vi "GV-GetLegendRange.vi"(8 "error in (no error)":errorcluster, 9 "Coords":T1, 11 "Gviewer in":refnum<class "Gviewer.lvclass">) -> (0 "error out":errorcluster, 1 "Where?":enum16{"Scroll over Plot", "Scroll over Legend"}(ring), 3 "Gviewer out":refnum<class "Gviewer.lvclass">)   [LabVIEW 2020, in "Sgraph_lib_V1.lvlib" / "Gviewer.lvclass"]
doc: "Andre Koelewijn, 25 April 2021\n\nCheck if the mouse is hovering over the Legend section or not"
uses:
  Gviewer.lvclass
  <vilib>/Utility/miscctls.llb/LVPoint32TypeDef.ctl
  Gviewer.lvclass/Gviewer.ctl
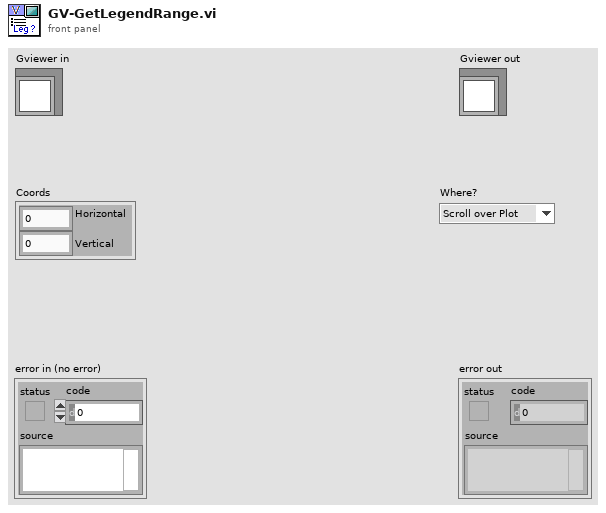
[diagram p1: front panel]
types:
  T1 = typedef "LVPoint32TypeDef.ctl" = cluster{"Horizontal":i32, "Vertical":i32}
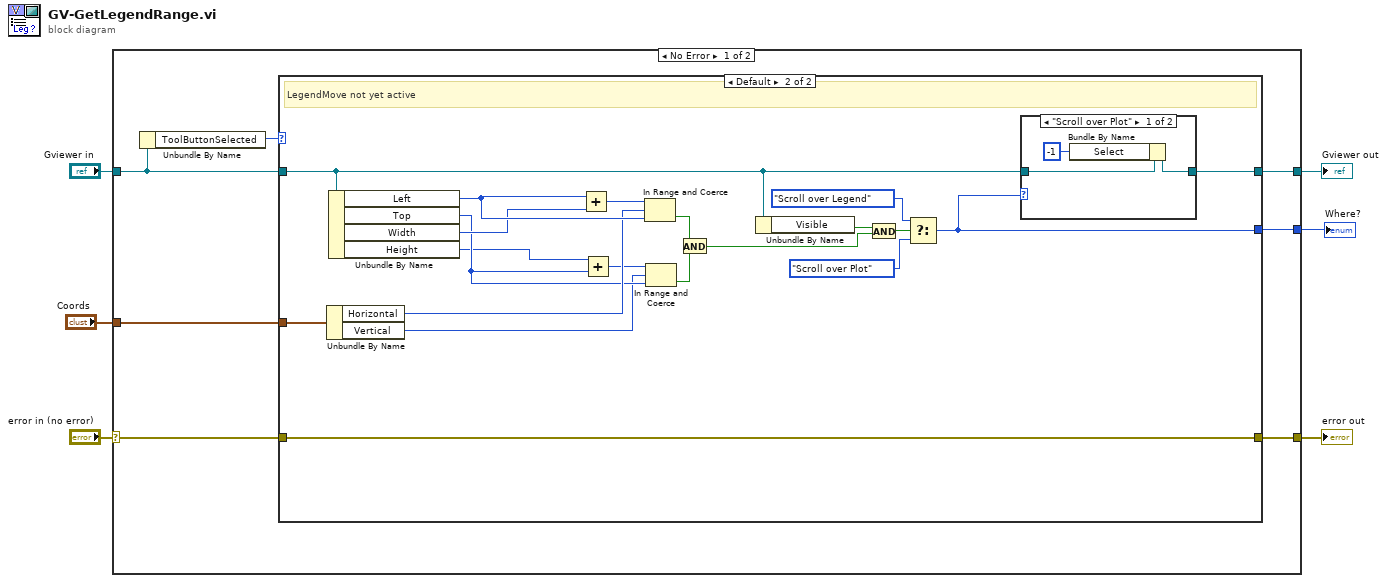
[diagram p0: block diagram]
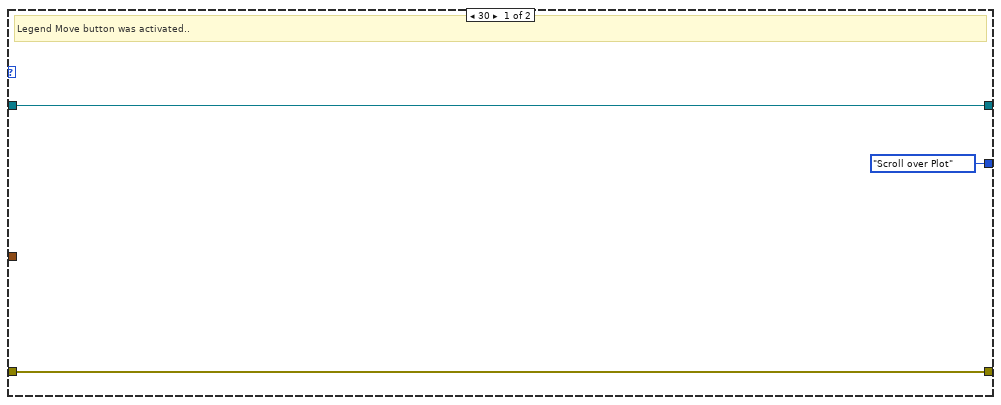
[diagram p2: hidden frame]
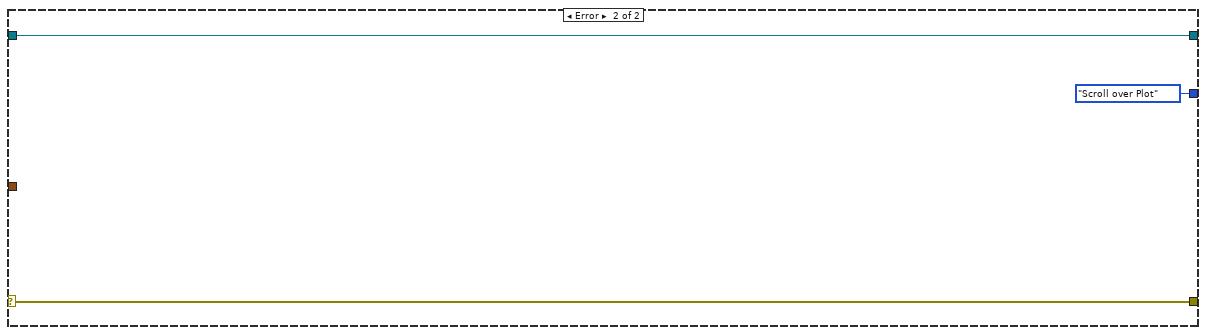
[diagram p4: hidden frame]
diagram:
  n1 = case shown="No Error" "error in (no error)" {
    selector: "error in (no error)" -> [w8 w43]
    tunnel: [w7 w43] -> w5
    tunnel: [w11 w42] -> w3
    tunnel: "Gviewer in" -> [w10 w42]
    tunnel: "Coords" -> [w13 _]
    tunnel: [w12 enum16{"Scroll over Plot", "Scroll over Legend"}."Scroll over Plot" ("Where?")] -> w1
    frame No Error {
      n2 = Unbundle By Name(w10) -> ("ToolButtonSelected"=w9:i32)
      n3 = case shown="Default" w9 {
        tunnel: w13 -> [_ w36]
        tunnel: [enum16{"Scroll over Plot", "Scroll over Legend"}."Scroll over Plot" ("Where?") w20] -> w12
        tunnel: [w16 w19] -> w11
        tunnel: w10 -> [w16 w18]
        tunnel: w8 -> [w15 w17]
        tunnel: [w15 w17] -> w7
        frame 30 {
          # "Legend Move button was activated.."
        }
        frame Default {
          # "LegendMove not yet active"
          n4 = Unbundle By Name(w36) -> ("Horizontal"=w32:i32, "Vertical"=w28:i32)
          n5 = Unbundle By Name(w18) -> ("Left"=w35:i32, "Top"=w31:i32, "Width"=w34:u32, "Height"=w30:u32)
          n6 = Add(x=w35, y=w34) -> (x+y=w33:u32)
          n7 = Add(x=w30, y=w31) -> (x+y=w29:u32)
          n8 = In Range and Coerce(upper limit=w33, x=w32, lower limit=w35) -> (In Range?=w27:bool)  [unwired: 1 out]
          n9 = In Range and Coerce(upper limit=w29, x=w28, lower limit=w31) -> (In Range?=w26:bool)  [unwired: 1 out]
          n10 = And(x=w27, y=w26) -> (x .and. y?=w24:bool)
          n11 = Unbundle By Name(w18) -> ("Visible"=w25:bool)
          n12 = And(x=w25, y=w24) -> (x .and. y?=w23:bool)
          n13 = Select(t=enum16{"Scroll over Plot", "Scroll over Legend"}."Scroll over Legend" ("Where?"), s=w23, f=enum16{"Scroll over Plot", "Scroll over Legend"}."Scroll over Plot" ("Where?")) -> (s? t:f=w20:enum16{"Scroll over Plot", "Scroll over Legend"})
          n14 = case shown="\"Scroll over Plot\"" w20 {
            tunnel: w18 -> [w39 w40]
            tunnel: [w38 w40] -> w19
            frame "Scroll over Plot" {
              n15 = Bundle By Name(cluster=w39, "Select"=-1 ("Legend.Select")) -> (w38:refnum<class "Gviewer.lvclass">)
            }
            frame "Scroll over Legend" {
            }
          }
        }
      }
    }
    frame Error {
    }
  }
  "error out" <- w5
  "Gviewer out" <- w3
  "Where?" <- w1
